vi "Build VIHelpeks Deployment.vi"() -> ()   [LabVIEW 2014]
doc: "::: VI Helpeks :::\nCopyright (c) 2000-2026 Konstantin Shifershteyn. All rights reserved."
panel:
  out "Excluded files":string
  in  "Exclude undesired paths":bool=TRUE caption="Exclude undesired files & folders"
  # "VI Helpeks\nCopyright (c) 2012-2026 Konstantin Shifershteyn"
  # "This VI generates VI Helpeks deployment, which is then used for creating a .VIP package."
  # "Before starting this VI, it is strongly recommended to close all VIs that use VI Helpeks VIs."
  # "Run this VI to generate VI Helpeks deployment, which are saved in the /__Deploy/ folder.\nThe deployment VIs are saved for both the running LabVIEW version and LabVIEW 2014. Both deployments\ninclude the necessary toolkit VIs and assets, and are ready for further distribution.\n\n\nBUILD  .VIP  PACKAGE\n\nTo build the VI Helpeks distribution package (.VIP), open the VI Helpeks (LV2014).vipb file\nin the VIPM Package Builder. This file uses the deployment for LabVIEW 2014 as the source."
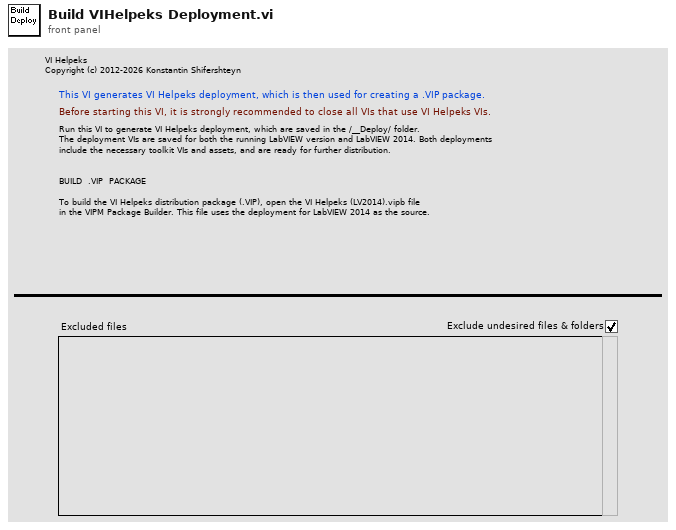
[diagram p1: front panel]
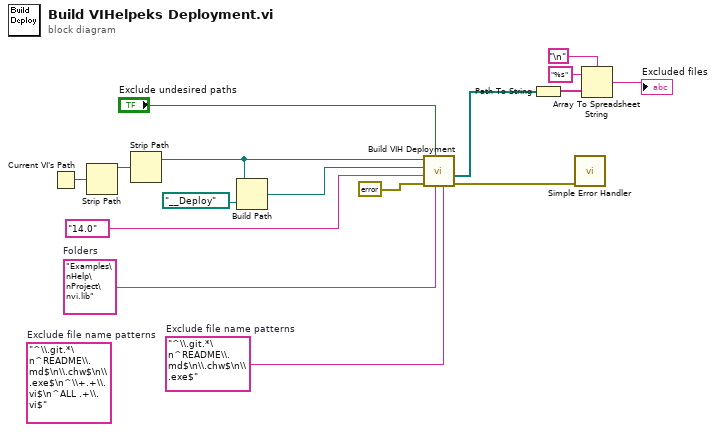
[diagram p0: block diagram]
diagram:
  (unwired) "^\\.git.*\n^README\\.md$\n\\.chw$\n\\.exe$\n^\\+.+\\.vi$\n^ALL .+\\.vi$"  # Exclude file name patterns
  w13 = "^\\.git.*\n^README\\.md$\n\\.chw$\n\\.exe$"  # Exclude file name patterns
  w16 = "Examples\nHelp\nProject\nvi.lib"  # Folders
  n1 = Current VI's Path() -> (path=w10:path)
  n2 = Strip Path(path=w10) -> (stripped path=w11:path)  [unwired: 1 out]
  n3 = Strip Path(path=w11) -> (stripped path=w8:path)  [unwired: 1 out]
  n4 = Build Path(base path=w8, name or relative path=path "__Deploy" ("Target Dir")) -> (appended path=w6:path)
  n5 = call "Build VIH Deployment.vi"("Exclude file name patterns"=w13, "Folders"=w16, "Exclude undesired paths (T)"="Exclude undesired paths", "error in"=errorcluster {"status"=FALSE, "code"=0, "source"=""}, "LV Version"="14.0", "Target Dir"=w6, "Source Dir"=w8) -> ("error out"=w9:errorcluster, "Excluded Paths"=w14:path[])  [unwired: 1 in, 2 out]
  n6 = Path To String(path=w14) -> (string=w4:string[])
  n7 = call <vilib>:"Simple Error Handler.vi"("error in (no error)"=w9) -> ()  [unwired: 4 in, 5 out]
  n8 = Array To Spreadsheet String(delimiter (Tab)="\n", array=w4, 3:"%s" ("format string")) -> (spreadsheet string=→"Excluded files":string)
